vi "VM Spy - context quick info (name+num).vi"(4 "handle":T1=-1) -> (1 "context info":string)   [LabVIEW 2021]
doc: "::: CalcExpress Toolkit :::\nCopyright (c) 2000-2026 Konstantin Shifershteyn. All rights reserved."
uses:
  vi.lib/addons/CalcExpress/cetypes.llb/VarMan Variable Context Handle.ctl
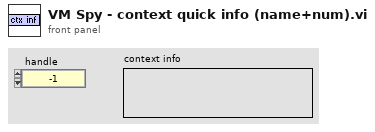
[diagram p1: front panel]
types:
  T1 = typedef "VarMan Variable Context Handle.ctl" = i32
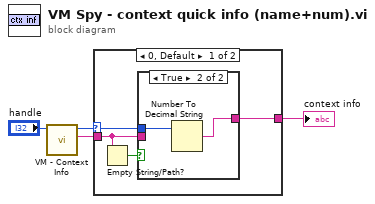
[diagram p0: block diagram]
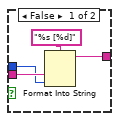
[diagram p2: hidden frame]
diagram:
  n1 = call "VM - Context Info.vi"("VC Handle"="handle") -> ("VC Name"=w4:string, "dup VC Handle"=w3:T1)  [unwired: 6 in, 3 out]
  n2 = case shown="0, Default" w3 {
    selector: w3 -> [w6 _]
    tunnel: [w7 w15] -> w1
    tunnel: w4 -> [w5 w15]
    frame 0, Default {
      n3 = Empty String/Path?(string/path=w5) -> (empty?=w8:bool)
      n4 = case shown="True" w8 {
        tunnel: [w11 w13] -> w7
        tunnel: w5 -> [w10 _]
        tunnel: w6 -> [w9 w14]
        frame False {
          n5 = Format Into String(format string="%s [%d]", w10, w9) -> (resulting string=w11:string)  [unwired: 2 in, 1 out]
        }
        frame True {
          n6 = Number To Decimal String(number=w14) -> (decimal integer string=w13:string)  [unwired: 1 in]
        }
      }
    }
    frame -1 {
    }
  }
  "context info" <- w1
